vi "order-analysis-block-test.vi"(1 "Order Settings":T1={"Pulses per Rev"=1, "Trigger Level (V)"=2.5, "Hysteresis (V)"=0.5, "Slope"=enum."Rising", "Revs per Spectrum"=16, "Min Valid RPM"=300.0, "Orders"=[1.0, 2.0, 3.57, 4.0, 24.0], "Band Half-Width (order)"=0.19, "Max Order"=64.0, "Phase Bandwidth (order)"=1.0}, 4 "Noise (g rms)":dbl=0.01, 5 "Phases (deg)":dbl[](array[numeric])=[30.0, 0.0, 0.0, 0.0, 0.0], 6 "Orders":dbl[](array[numeric])=[1.0, 2.0, 3.57, 4.0, 24.0], 7 "Amplitudes (g pk)":dbl[](array[numeric])=[0.5, 0.2, 0.1, 0.05, 0.3], 8 "error in (no error)":errorcluster, 9 "Duration (s)":dbl=30.0, 10 "Ramps":T2(array[cluster]), 11 "Base RPM":dbl=3000.0) -> (0 "error out":errorcluster, 2 "True RPM":dbl[](array[numeric]), 3 "Values":dbl[][](array[numeric]))   [LabVIEW 2026]
doc: "Unit-test harness for OrderAnalysis.vi. Synthesises accel (sum of order sines, peak amplitudes, uniform noise) and a 1 ppr 0-5 V square tach (rising edge at shaft angle 0) for rpm(t) = Base RPM + sum of linear ramps, cuts it into 0.1 s blocks (5120 S @ 51.2 kS/s) and calls OrderAnalysis.vi block by block like FlexLogger Process.vi does (reset? TRUE on block 0, state in a shift register). Returns NUMERIC arrays only: Values [blocks x 12] in OrderAnalysis channel order, True RPM at each block centre."
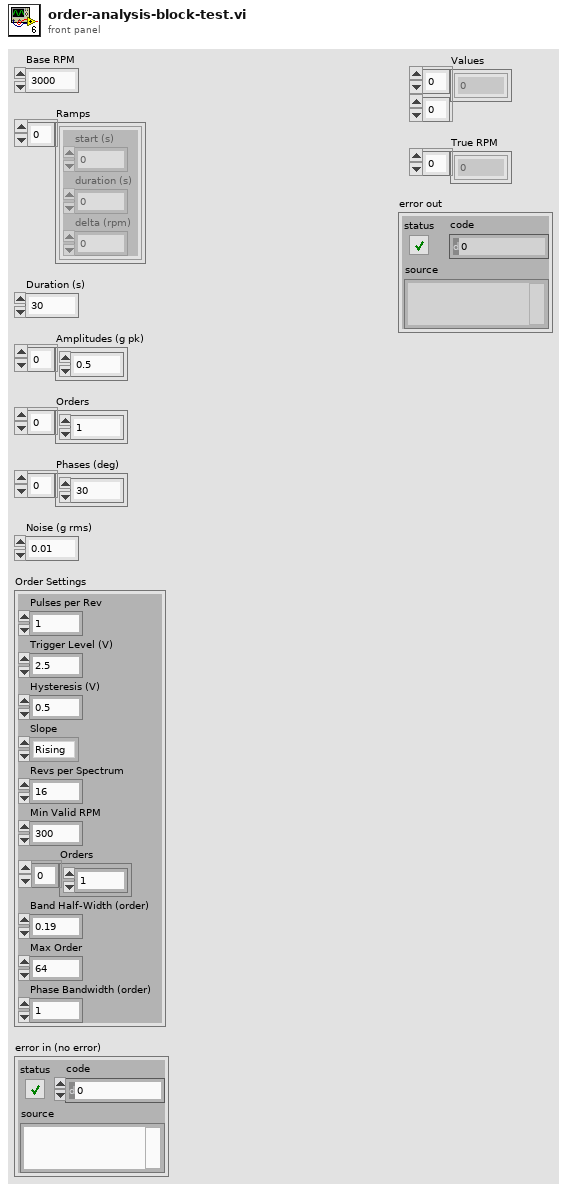
[diagram p1: front panel]
types:
  T1 = cluster{"Pulses per Rev":i32, "Trigger Level (V)":dbl, "Hysteresis (V)":dbl, "Slope":enum16{"Rising", "Falling"}, "Revs per Spectrum":i32, "Min Valid RPM":dbl, "Orders":dbl[], "Band Half-Width (order)":dbl, "Max Order":dbl, "Phase Bandwidth (order)":dbl}
  T2 = cluster{"start (s)":dbl, "duration (s)":dbl, "delta (rpm)":dbl}[]
  T3 = cluster{"Sample Count":dbl, "Last Time":dbl, "Last RPM":dbl, "Prev Time":dbl, "Prev RPM":dbl, "Anchor Time":dbl, "Anchor RPM":dbl, "RPM Rate":dbl, "Held Values":dbl[], "Has Spectrum":bool, "Was Valid":bool, "Acc SumSq":dbl, "Acc N":dbl}
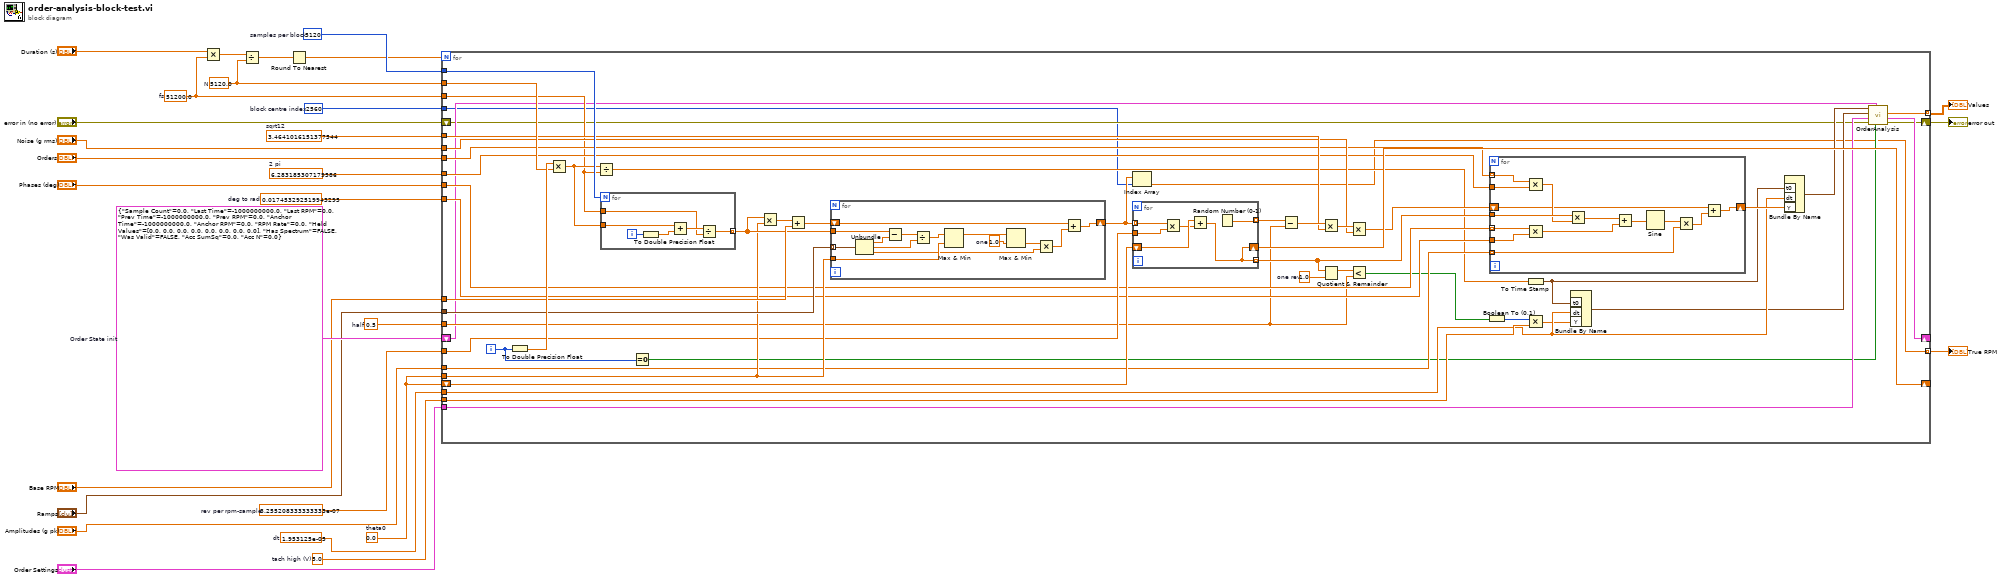
[diagram p0: block diagram]
diagram:
  w6 = 2560  # block centre index
  w7 = 5.0  # tach high (V)
  w8 = 6.283185307179586  # 2 pi
  w9 = 0.017453292519943295  # deg to rad
  w10 = 0.5  # half
  w11 = 3.4641016151377544  # sqrt12
  w12 = 1.953125e-05  # dt
  w13 = 3.255208333333333e-07  # rev per rpm-sample
  w5 = 0.0  # theta0
  w25 = T3 {"Sample Count"=0.0, "Last Time"=-1000000000.0, "Last RPM"=0.0, "Prev Time"=-1000000000.0, "Prev RPM"=0.0, "Anchor Time"=-1000000000.0, "Anchor RPM"=0.0, "RPM Rate"=0.0, "Held Values"=[0.0, 0.0, 0.0, 0.0, 0.0, 0.0, 0.0, 0.0], "Has Spectrum"=FALSE, "Was Valid"=FALSE, "Acc SumSq"=0.0, "Acc N"=0.0}  # Order State init
  w14 = 5120.0  # N
  w15 = 5120  # samples per block
  w16 = 51200.0  # fs
  n1 = Multiply(x="Duration (s)", y=w16) -> (x*y=w27:dbl)
  n2 = Divide(x=w27, y=w14) -> (x/y=w26:dbl)
  n3 = Round To Nearest(number=w26) -> (nearest integer value=w4:dbl)
  n4 = for {
    N: w4 -> [_]
    shift-right: [w68] -> _
    shift-left: w5 -> [w67]
    shift-right: [w35] -> _
    shift-left: w25 -> [w38]
    shift-right: [w34] -> w1
    shift-left: "error in (no error)" -> [w36]
    tunnel: "Base RPM" -> [w74]
    tunnel: "Ramps" -> [w73]
    tunnel: "Amplitudes (g pk)" -> [w60]
    tunnel: "Orders" -> [w61]
    tunnel: "Phases (deg)" -> [w59]
    tunnel: "Noise (g rms)" -> [w62]
    tunnel: "Order Settings" -> [w39]
    tunnel: w16 -> [w47]
    tunnel: w15 -> [w76]
    tunnel: w14 -> [w77]
    tunnel: w13 -> [w69]
    tunnel: w12 -> [w43]
    tunnel: w11 -> [w64]
    tunnel: w10 -> [w52]
    tunnel: w9 -> [w57]
    tunnel: w8 -> [w58]
    tunnel: w7 -> [w49]
    tunnel: w6 -> [w32]
    tunnel: w5 -> [w71]
    tunnel: [w31] -> w3 mode=indexing
    tunnel: [w30] -> w2 mode=indexing
    i -> [w29]
    w54 = 1.0  # one rev
    n5 = To Double Precision Float(number=w29) -> (double precision float=w78:dbl)
    n6 = Multiply(x=w78, y=w77) -> (x*y=w48:dbl)
    n7 = Divide(x=w48, y=w47) -> (x/y=w46:dbl)
    n8 = for {
      N: w76 -> [_]
      tunnel: w48 -> [w118]
      tunnel: w47 -> [w115]
      tunnel: [w114] -> w72 mode=indexing
      i -> [w113]
      n9 = To Double Precision Float(number=w113) -> (double precision float=w117:dbl)
      n10 = Add(x=w118, y=w117) -> (x+y=w116:dbl)
      n11 = Divide(x=w116, y=w115) -> (x/y=w114:dbl)
    }
    n12 = Equal To 0?(x=w29) -> (x = 0?=w37:bool)
    n13 = Multiply(x=w72, y=w71) -> (x*y=w75:dbl[])
    n14 = Add(x=w75, y=w74) -> (x+y=w70:dbl[])
    n15 = for {
      tunnel: w73 -> [w112] mode=indexing
      tunnel: w72 -> [w111]
      tunnel: w71 -> [w106]
      shift-right: [w99] -> w33
      shift-left: w70 -> [w101]
      w104 = 1.0  # one
      n16 = Unbundle(w112) -> ("start (s)"=w110:dbl, "duration (s)"=w108:dbl, "delta (rpm)"=w102:dbl)
      n17 = Subtract(x=w111, y=w110) -> (x-y=w109:dbl[])
      n18 = Divide(x=w109, y=w108) -> (x/y=w107:dbl[])
      n19 = Max & Min(x=w107, y=w106) -> (max(x,y)=w105:dbl[])  [unwired: 1 out]
      n20 = Max & Min(x=w105, y=w104) -> (min(x,y)=w103:dbl[])  [unwired: 1 out]
      n21 = Multiply(x=w103, y=w102) -> (x*y=w100:dbl[])
      n22 = Add(x=w101, y=w100) -> (x+y=w99:dbl[])
    }
    n23 = Index Array(array=w33, index=w32) -> (element=w30:dbl)
    n24 = for {
      tunnel: w33 -> [w98] mode=indexing
      tunnel: w69 -> [w97]
      shift-right: [w94] -> w68
      shift-left: w67 -> [w96]
      tunnel: [w94] -> w55 mode=indexing
      tunnel: [w93] -> w66 mode=indexing
      n25 = Multiply(x=w98, y=w97) -> (x*y=w95:dbl)
      n26 = Add(x=w96, y=w95) -> (x+y=w94:dbl)
      n27 = Random Number (0-1)() -> (number: 0 to 1=w93:dbl)
    }
    n28 = Subtract(x=w66, y=w52) -> (x-y=w65:dbl[])
    n29 = Multiply(x=w65, y=w64) -> (x*y=w63:dbl[])
    n30 = Quotient & Remainder(x=w55, y=w54) -> (x-y*floor(x/y)=w53:dbl[])  [unwired: 1 out]
    n31 = Multiply(x=w63, y=w62) -> (x*y=w56:dbl[])
    n32 = Less?(x=w53, y=w52) -> (x < y?=w51:bool[])
    n33 = Boolean To (0,1)(Boolean=w51) -> (0, 1=w50:i16[])
    n34 = for {
      tunnel: w61 -> [w92] mode=indexing
      tunnel: w60 -> [w82] mode=indexing
      tunnel: w59 -> [w88] mode=indexing
      tunnel: w55 -> [w90]
      tunnel: w58 -> [w91]
      tunnel: w57 -> [w87]
      shift-right: [w79] -> w45
      shift-left: w56 -> [w81]
      n35 = Multiply(x=w92, y=w91) -> (x*y=w89:dbl)
      n36 = Multiply(x=w88, y=w87) -> (x*y=w85:dbl)
      n37 = Multiply(x=w90, y=w89) -> (x*y=w86:dbl[])
      n38 = Add(x=w86, y=w85) -> (x+y=w84:dbl[])
      n39 = Sine(x=w84) -> (sin(x)=w83:dbl[])
      n40 = Multiply(x=w83, y=w82) -> (x*y=w80:dbl[])
      n41 = Add(x=w81, y=w80) -> (x+y=w79:dbl[])
    }
    n42 = Multiply(x=w50, y=w49) -> (x*y=w42:dbl[])
    n43 = To Time Stamp(1:w46) -> (0:w44:timestamp)
    n44 = Bundle By Name("t0"=w44, "dt"=w43, "Y"=w42) -> (w40:waveform(dbl))  [unwired: 1 in]
    n45 = Bundle By Name("t0"=w44, "dt"=w43, "Y"=w45) -> (w41:waveform(dbl))  [unwired: 1 in]
    n46 = call "OrderAnalysis.vi"("reset? (F)"=w37, "Order State in"=w38, "error in (no error)"=w36, "Order Settings"=w39, "Tach In"=w40, "Accel In"=w41) -> ("error out"=w34:errorcluster, "Order State out"=w35:T3, "Order Values"=w31:dbl[])  [unwired: 2 in, 1 out]
  }
  "Values" <- w3
  "True RPM" <- w2
  "error out" <- w1
